vi "Inspect Queue Items.vi"(8 "error in (no error)":errorcluster, 11 "Message Enqueuer in":refnum<class "Message Enqueuer.lvclass">) -> (0 "error out":errorcluster, 1 "Message Names":string[](array[string]), 2 "# Messages in queue":i32, 3 "Message Enqueuer out":refnum<class "Message Enqueuer.lvclass">)   [LabVIEW 2020, in "Actor Framework.lvlib" / "Message Enqueuer.lvclass"]
doc: "This VI can be used to inspect the Actor Queue.\n\nTo protect the actor functionality it show information about the queue but can not change it.\n\nReturns:\n# of Messages in queue - Current queue ellement count for the Actor.\nThis can be useful for seeing if your processing is causing the queue to fill up helping you to better architect your methods.\n- Message Names (Array of Strings) - Names of Each Message Class in the queue. \nThis is helpful for bug fixing or tracking cross message errors etc.\nString names are returned rather than message lvclasses to prevent users from interfering with the payload of the message causing possible actor system problems."
uses:
  Message Enqueuer.lvclass
  Message Enqueuer.lvclass/Message Enqueuer.ctl
  Message Priority Queue/Message Priority Queue.lvclass
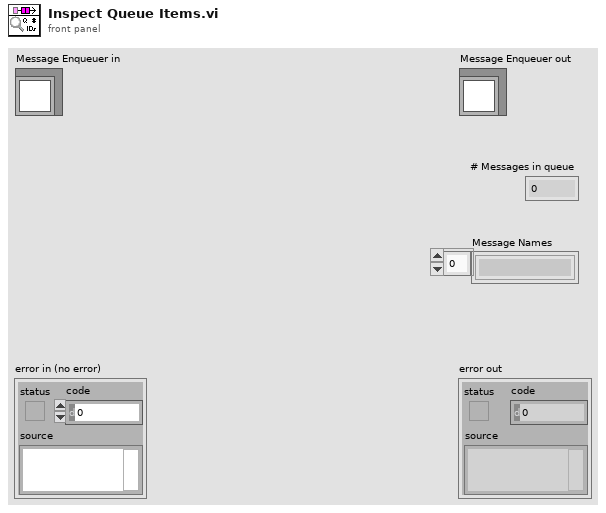
[diagram p1: front panel]
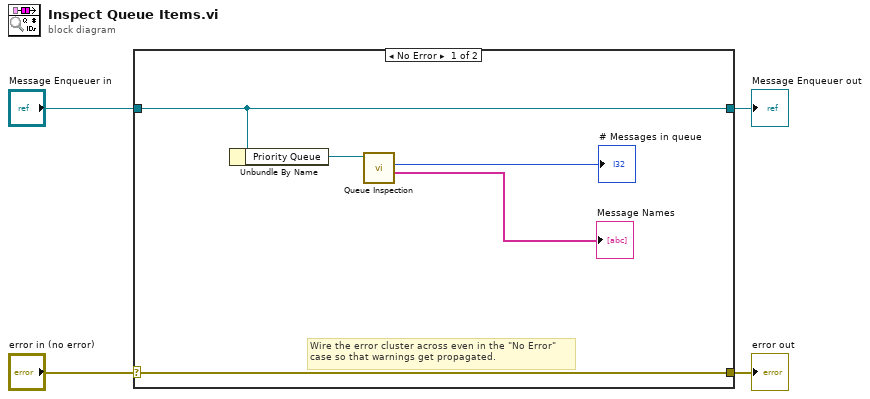
[diagram p0: block diagram]
diagram:
  n1 = case shown="No Error" "error in (no error)" {
    selector: "error in (no error)" -> [w9 w11]
    tunnel: [w9 w11] -> w3
    tunnel: [w8 w10] -> w1
    tunnel: "Message Enqueuer in" -> [w8 w10]
    frame No Error {
      # "Wire the error cluster across even in the \"No Error\"\ncase so that warnings get propagated."
      n2 = Unbundle By Name(w8) -> ("Priority Queue"=w7:refnum<class "Message Priority Queue.lvclass">)
      n3 = call "Queue Inspection.vi"("Priority Queue in"=w7) -> ("Element Names"=→"Message Names":string[], "# elements in queue"=→"# Messages in queue":i32)  [unwired: 7 in, 2 out]
    }
    frame Error {
    }
  }
  "error out" <- w3
  "Message Enqueuer out" <- w1
